vi "Is Theory.vi"(11 "ProjectItem Refnum":refnum<vi>) -> (2 "Is Theory":bool, 3 "Json File":path)   [LabVIEW 2017, in "LVUnit Test Discoverer.lvclass"]
uses:
  LVUnit Test Discoverer.lvclass
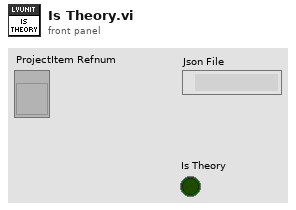
[diagram p1: front panel]
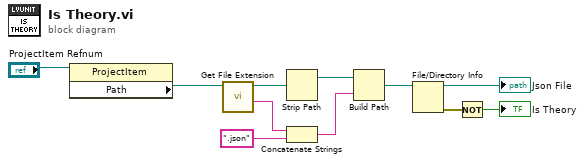
[diagram p0: block diagram]
diagram:
  n1 = property class="ProjectItem"(reference="ProjectItem Refnum") -> ("Path"=w10:path)  [unwired: 1 in, 2 out]
  n2 = call <vilib>:"Get File Extension.vi"("file"=w10) -> ("filename without extension"=w6:string, "dup file"=w9:path)  [unwired: 6 in, 3 out]
  n3 = Strip Path(path=w9) -> (stripped path=w8:path)  [unwired: 1 out]
  n4 = Concatenate Strings(w6, ".json") -> (w5:string)
  n5 = Build Path(base path=w8, name or relative path=w5) -> (appended path=w4:path)
  n6 = File/Directory Info(path=w4) -> (path out=→"Json File":path, error out=w3:errorcluster)  [unwired: 1 in, 5 out]
  n7 = Not(x=w3) -> (.not. x?=→"Is Theory":bool)
